vi "init Self Alignment.vi"(8 "error in (no error)":errorcluster, 11 "FSV-40N in":refnum<class "FSV-40N.lvclass">) -> (0 "error out":errorcluster, 3 "FSV-40N out":refnum<class "FSV-40N.lvclass">)   [LabVIEW 2023, in "Spectrum Analyzer.lvlib" / "FSV-40N.lvclass"]
uses:
  FSV-40N.lvclass
  FSV-40N.lvclass/FSV-40N.ctl
  Spectrum Analyzer.lvlib
  <vilib>/ErrorRing/Error Ring.xnode
  <vilib>/Utility/error.llb/Error Cluster From Error Code.vi
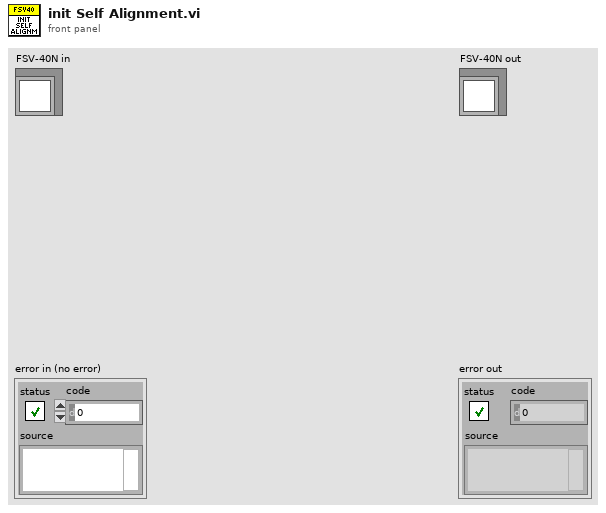
[diagram p1: front panel]
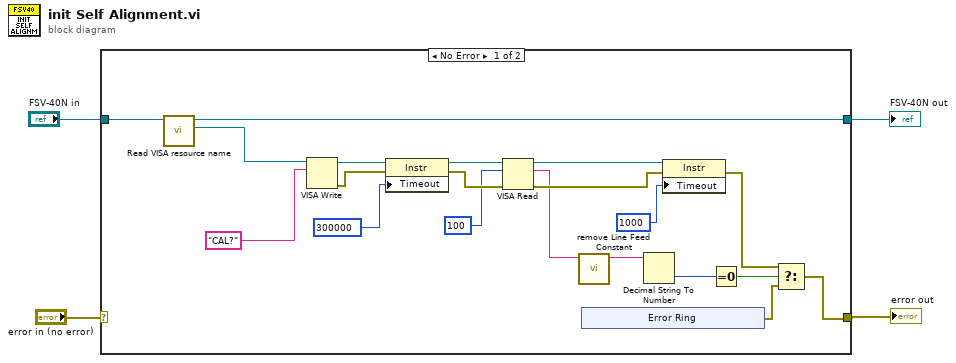
[diagram p0: block diagram]
diagram:
  n1 = case shown="No Error" "error in (no error)" {
    selector: "error in (no error)" -> [_ w30]
    tunnel: "FSV-40N in" -> [w24 w31]
    tunnel: [w22 w31] -> w3
    tunnel: [w5 w30] -> w1
    frame No Error {
      n2 = call "Read VISA resource name.vi"("FSV-40N in"=w24) -> ("VISA resource name"=w23:refnum<visa-resource-name>, "FSV-40N out"=w22:refnum<class "FSV-40N.lvclass">)  [unwired: 8 in, 1 out]
      n3 = VISA Write(VISA resource name=w23, write buffer="CAL?") -> (VISA resource name out=w20:refnum<visa-resource-name>, error out=w18:errorcluster)  [unwired: 1 in, 1 out]
      n4 = property class="Instr"(reference=w20, error in=w18, "Timeout"=u32 300000 ("General Settings:Timeout Value")) -> (reference out=w17:refnum<visa-resource-name>, error out=w16:errorcluster)
      n5 = VISA Read(VISA resource name=w17, byte count=u32 100, error in (no error)=w16) -> (VISA resource name out=w14:refnum<visa-resource-name>, read buffer=w11:string, error out=w13:errorcluster)  [unwired: 1 out]
      n6 = call "remove Line Feed Constant.vi"("Input String"=w11) -> ("Line Feed Removed String"=w10:string)  [unwired: 10 in]
      n7 = xnode "Error Ring"() -> ("error out"=w6:errorcluster)
      n8 = Decimal String To Number(string=w10) -> (number=w9:i32)  [unwired: 2 in, 1 out]
      n9 = property class="Instr"(reference=w14, error in=w13, "Timeout"=u32 1000 ("General Settings:Timeout Value")) -> (error out=w7:errorcluster)  [unwired: 1 out]
      n10 = Equal To 0?(x=w9) -> (x = 0?=w8:bool)
      n11 = Select(t=w7, s=w8, f=w6) -> (s? t:f=w5:errorcluster)
    }
    frame Error {
    }
  }
  "error out" <- w1
  "FSV-40N out" <- w3
